vi "GV_ToolbarDiskType.vi"(7 "Layer":i32, 8 "Hor-pos":i32, 11 "Pict in":picture) -> (0 "x":i16, 1 "y":i16, 3 "Pict out":picture)   [LabVIEW 2020, in "Sgraph_lib_V1.lvlib" / "Gviewer.lvclass"]
doc: "Andre Koelewijn, 20 June 2021\n\nDraw the Memory or Disk icon & memory Layer into the toolbar"
uses:
  Gviewer.lvclass
  <vilib>/picture/picture.llb/imagedata.ctl
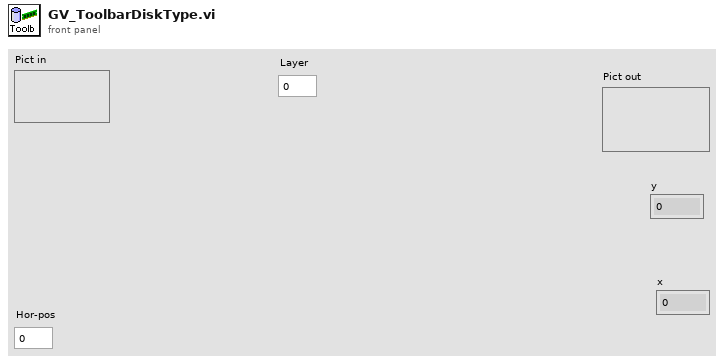
[diagram p1: front panel]
types:
  T1 = cluster{"horizontal":enum16{"left", "center", "right"}, "vertical":enum16{"top", "center", "bottom"}}
  T2 = typedef "imagedata.ctl" = cluster{"image type":i32, "image depth":i32, "image":u8[], "mask":u8[], "colors":u32[], "Rectangle":cluster{"left":i16, "top":i16, "right":i16, "bottom":i16}}
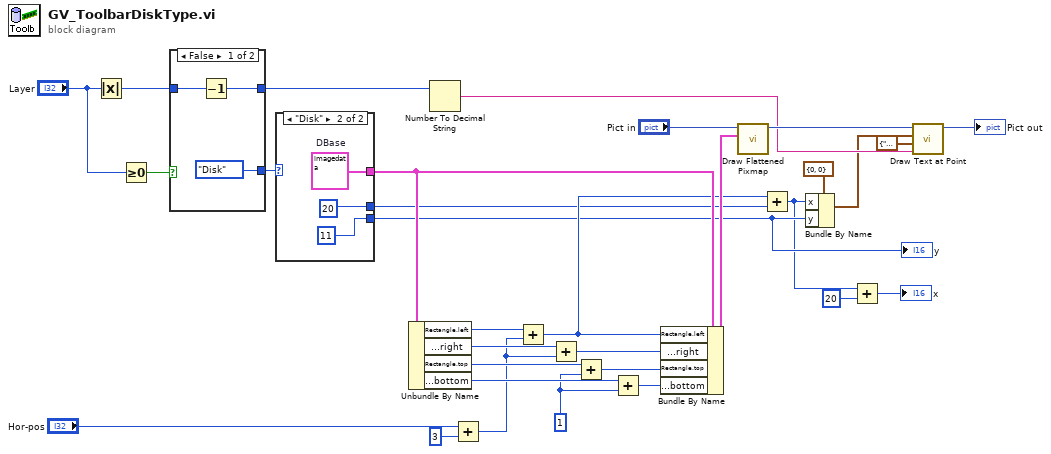
[diagram p0: block diagram]
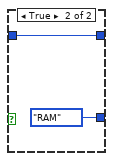
[diagram p2: hidden frame]
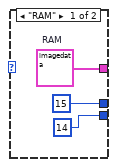
[diagram p3: hidden frame]
diagram:
  w23 = 1
  n1 = Absolute Value(x="Layer") -> (abs(x)=w5:i32)
  n2 = Greater Or Equal To 0?(x="Layer") -> (x >= 0?=w16:bool)
  n3 = case shown="False" w16 {
    tunnel: [enum16{"RAM", "Disk"}."Disk" ("MemoryType") enum16{"RAM", "Disk"}."RAM" ("MemoryType")] -> w17
    tunnel: w5 -> [w33 w35]
    tunnel: [w32 w35] -> w4
    frame False {
      n4 = Decrement(x=w33) -> (x-1=w32:i32)
    }
    frame True {
    }
  }
  n5 = case shown="\"Disk\"" w17 {
    tunnel: [w39 w42] -> w29
    tunnel: [i16 14 ("y") i16 11 ("y")] -> w7
    tunnel: [15 ("y") 20 ("y")] -> w6
    frame "RAM" {
      w39 = T2 {"image type"=0, "image depth"=32, "image"=array[3360 elements], "mask"=[0, 0, 0, 0, 4, 8, 32, 128, 14, 28, 113, 192, 14, 28, 113, 192, 14, 28, 113, 192, 63, 255, 255, 240, 127, 255, 255, 248, 127, 255, 255, 248, 127, 255, 255, 248, 127, 255, 255, 248, 127, 255, 255, 248, 127, 255, 255, 248, 127, 255, 255, 248, 127, 255, 255, 248, 127, 255, 255, 248, 127, 255, 255, 248, 127, 255, 255, 248, 127, 255, 255, 248, 127, 255, 255, 248, 127, 255, 255, 248, 127, 255, 255, 248, 127, 255, 255, 248, 63, 255, 255, 240, 14, 56, 227, 128, 14, 56, 227, 128, 14, 56, 227, 128, 4, 16, 65, 0, 0, 0, 0, 0], "colors"=[], "Rectangle"={"left"=0, "top"=0, "right"=30, "bottom"=28}}  # RAM
    }
    frame "Disk" {
      w42 = T2 {"image type"=0, "image depth"=32, "image"=array[3472 elements], "mask"=[0, 0, 0, 0, 15, 255, 255, 192, 16, 0, 0, 48, 32, 0, 0, 16, 33, 240, 0, 8, 35, 248, 0, 8, 39, 252, 0, 8, 39, 252, 0, 8, 39, 252, 0, 8, 39, 252, 0, 8, 39, 252, 0, 8, 39, 252, 0, 8, 39, 252, 0, 8, 39, 252, 0, 8, 39, 252, 0, 8, 35, 248, 0, 8, 33, 240, 0, 8, 32, 0, 0, 16, 24, 0, 0, 48, 7, 255, 255, 192, 0, 1, 0, 0, 0, 1, 0, 0, 0, 3, 128, 0, 0, 4, 64, 0, 63, 252, 127, 248, 0, 4, 64, 0, 0, 3, 128, 0, 0, 0, 0, 0], "colors"=[], "Rectangle"={"left"=0, "top"=0, "right"=31, "bottom"=28}}  # DBase
    }
  }
  "y" <- w7
  n6 = Unbundle By Name(w29) -> ("Rectangle.left"=w31:i16, "Rectangle.right"=w30:i16, "Rectangle.top"=w26:i16, "Rectangle.bottom"=w24:i16)
  n7 = Number To Decimal String(number=w4) -> (decimal integer string=w12:string)  [unwired: 1 in]
  n8 = Add(x="Hor-pos", y=3) -> (x+y=w18:i32)
  n9 = Add(x=w31, y=w18) -> (x+y=w8:i32)
  n10 = Add(x=w30, y=w18) -> (x+y=w27:i32)
  n11 = Add(x=w26, y=w23) -> (x+y=w25:i32)
  n12 = Add(x=w24, y=w23) -> (x+y=w22:i32)
  n13 = Bundle By Name(cluster=w29, "Rectangle.left"=w8, "Rectangle.right"=w27, "Rectangle.top"=w25, "Rectangle.bottom"=w22) -> (w28:T2)
  n14 = call <vilib>:"Draw Flattened Pixmap.vi"("image data"=w28, "picture"="Pict in") -> ("new picture"=w15:picture)  [unwired: 7 in]
  n15 = Add(x=w8, y=w6) -> (x+y=w3:i32)
  n16 = Bundle By Name(cluster=cluster{"x":i16, "y":i16} {"x"=0, "y"=0} ("origin"), "x"=w3, "y"=w7) -> (w9:cluster{"x":i16, "y":i16})
  n17 = Add(x=w3, y=20) -> (x+y=→"x":i32)
  n18 = call <vilib>:"Draw Text at Point.vi"("text"=w12, "alignment(left, top)"=T1 {"horizontal"=enum."center", "vertical"=enum."center"}, "origin"=w9, "picture"=w15) -> ("new picture"=→"Pict out":picture)  [unwired: 6 in, 1 out]
